vi "test Switch Modules To Scan Mode.vi"(8 "error in (no error)":errorcluster, 11 "TestCase in":refnum<class "Scan Engine cRIO 904x-905x System Tests.lvclass">) -> (0 "error out":errorcluster, 3 "TestCase out":refnum<class "Scan Engine cRIO 904x-905x System Tests.lvclass">)   [LabVIEW 2016, in "Scan Engine cRIO 904x-905x System Tests.lvclass"]
uses:
  Scan Engine cRIO 904x-905x System Tests.lvclass
  <vilib>/nisyscfg/Filter Mode.ctl
  <vilib>/nisyscfg/Save Changes (Hardware).vi
  <vilib>/nisyscfg/Close (Filter).vi
  <vilib>/nisyscfg/Close (System).vi
  <vilib>/nisyscfg/Close (Resources).vi
  <vilib>/addons/_JKI Toolkits/VI Tester/TestCase.llb/TestCase.lvclass
  <vilib>/nisyscfg/nisyscfg.lvlib
  <resource>/objmgr/nisysapi.rc
  <resource>/objmgr/nicriosae.rc
  C:/Program Files (x86)/National Instruments/LabVIEW 2016/vi.lib/addons/_JKI Toolkits/VI Tester/TestCase.llb/TestCase.lvclass
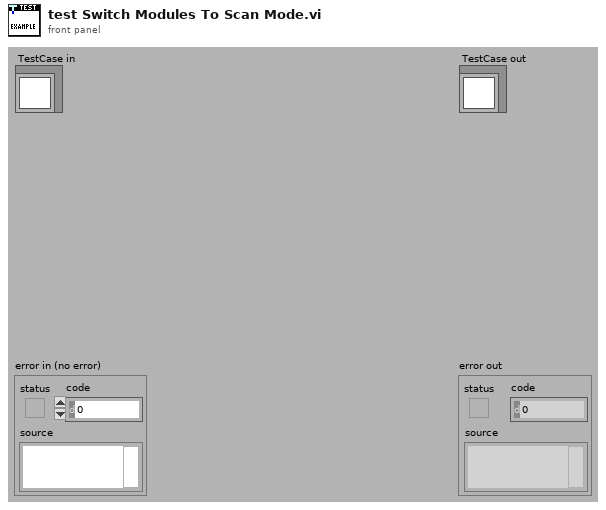
[diagram p1: front panel]
types:
  T1 = cluster{"y":i32, "Devices & Chassis:Bus Specific:cRIO Module Programming Mode":u32}[]
  T2 = typedef "nisyscfg.lvlib/Filter Mode.ctl" = i32
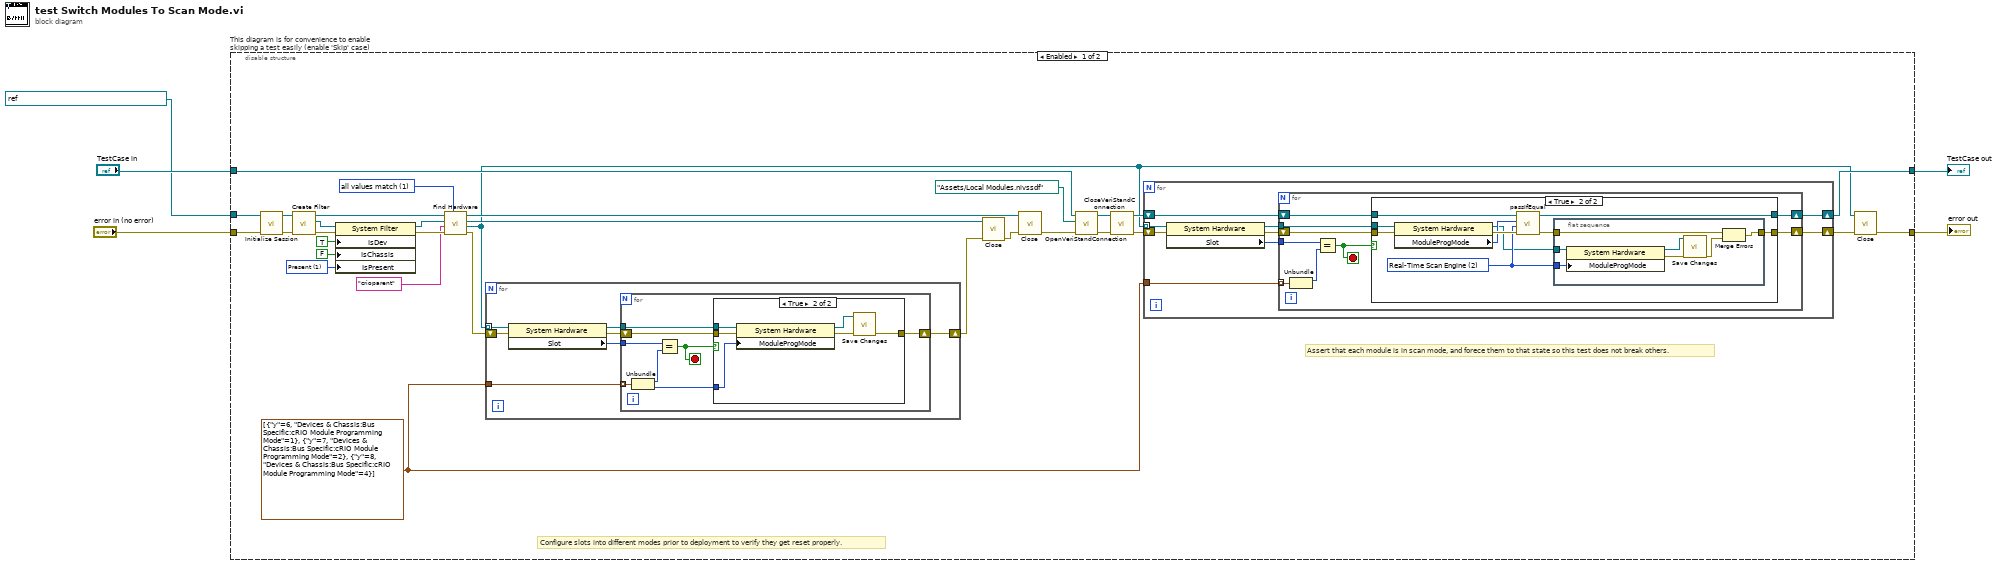
[diagram p0: block diagram]
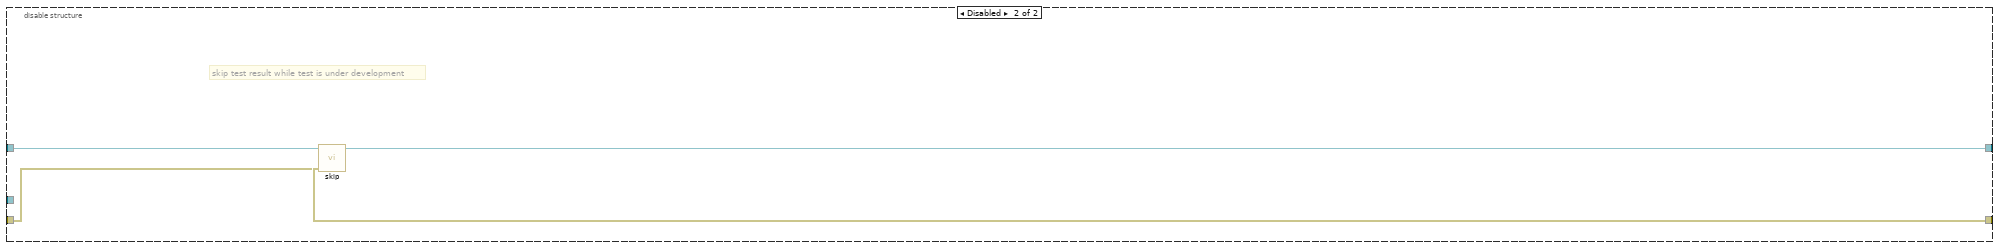
[diagram p4: hidden frame]
diagram:
  n1 = disable-structure "This diagram is for convenience to enable skipping a test easily (enable 'Skip' case)" shown="Enabled" {
    disable-tunnel: "TestCase in" -> [w17 w99]
    disable-tunnel: [w9 w97] -> w2
    disable-tunnel: [w7 w98] -> w4
    disable-tunnel: "error in (no error)" -> [w36 w96]
    disable-tunnel: refnum<k21> "NI-cRIO-9045-01CEEDFB (10.2.64.28)" ("Target (localhost)") -> [w26 _]
    frame Enabled {
      w12 = T1 [{"y"=6, "Devices & Chassis:Bus Specific:cRIO Module Programming Mode"=1}, {"y"=7, "Devices & Chassis:Bus Specific:cRIO Module Programming Mode"=2}, {"y"=8, "Devices & Chassis:Bus Specific:cRIO Module Programming Mode"=4}] ("output cluster")
      w22 = 1 items=["Initializing"=-2, "Unknown"=-1, "Not Present"=0, "Present"=1] ("Devices & Chassis:Is Present")
      w27 = T2 1 items=["all values match"=1, "any value matches"=2, "values do not match"=3, "all properties exist"=4] ("filter mode (all values match)")
      # "Configure slots into different modes prior to deployment to verify they get reset properly."
      # "Assert that each module is in scan mode, and forece them to that state so this test does not break others."
      n2 = call <vilib>:"Initialize Session.vi"("error in (no error)"=w36, "Target (localhost)"=w26) -> ("error out"=w28:errorcluster, "Session out"=w29:refnum<k21>)  [unwired: 8 in]
      n3 = call <vilib>:"Create Filter.vi"("error in (no error)"=w28, "Session in"=w29) -> ("error out"=w35:errorcluster, "Filter out"=w34:refnum<k20>, "Session out"=w33:refnum<k21>)  [unwired: 7 in]
      n4 = property class="System Filter"(reference=w34, error in=w35, "IsDev"=TRUE ("Is Chassis"), "IsChassis"=FALSE ("Is Chassis"), "IsPresent"=w22) -> (reference out=w31:refnum<k20>, error out=w32:errorcluster)
      n5 = call <vilib>:"Find Hardware.vi"("Filter Mode (all values match)"=w27, "error in (no error)"=w32, "Experts"="crioparent", "Filter in"=w31, "Session in"=w33) -> ("error out"=w21:errorcluster, "Resources out"=w6:refnum<k20>[], "Filter out"=w25:refnum<k20>, "Session out"=w19:refnum<k21>)  [unwired: 3 out]
      n6 = for {
        tunnel: w6 -> [w42] mode=indexing
        shift-right: [w37] -> w20
        shift-left: w21 -> [w43]
        tunnel: w12 -> [w40]
        n7 = property class="System Hardware"(reference=w42, error in=w43) -> (reference out=w39:refnum<k20>, error out=w38:errorcluster, "Slot"=w41:i32)
        n8 = for {
          tunnel: w41 -> [w51]
          tunnel: w40 -> [w50] mode=indexing
          tunnel: w39 -> [w47]
          shift-right: [w45] -> w37
          shift-left: w38 -> [w46]
          stop <- w44 stop-if-true
          n9 = Unbundle(w50) -> ("y"=w49:i32, "Devices & Chassis:Bus Specific:cRIO Module Programming Mode"=w48:u32)
          n10 = Equal?(x=w51, y=w49) -> (x = y?=w44:bool)
          n11 = case shown="True" w44 {
            tunnel: w48 -> [_ w58]
            tunnel: w47 -> [_ w57]
            tunnel: w46 -> [w52 w56]
            tunnel: [w52 w53] -> w45
            frame False {
            }
            frame True {
              n12 = property class="System Hardware"(reference=w57, error in=w56, "ModuleProgMode"=w58) -> (reference out=w55:refnum<k20>, error out=w54:errorcluster)
              n13 = call-poly <vilib>:"Save Changes.vi"("error in (no error)"=w54, "Resource in"=w55) -> ("error out"=w53:errorcluster)  [unwired: 6 in, 3 out]
            }
          }
        }
      }
      n14 = call-poly <vilib>:"Close.vi"("error in (no error)"=w20, "Filter in"=w25) -> ("error out"=w18:errorcluster)  [unwired: 9 in]
      n15 = call-poly <vilib>:"Close.vi"("error in (no error)"=w18, "Session in"=w19) -> ("error out"=w16:errorcluster)  [unwired: 9 in]
      n16 = call-dynamic "OpenVeriStandConnection.vi"("error in (no error)"=w16, "System Definition File"=path "Assets/Local Modules.nivssdf", "VeriStand Test Case in"=w17) -> ("error out"=w14:errorcluster, "VeriStand Test Case out"=w15:refnum<class "Scan Engine cRIO 904x-905x System Tests.lvclass">)  [unwired: 7 in]
      n17 = call-dynamic "CloseVeriStandConnection.vi"("error in (no error)"=w14, "VeriStand Test Case in"=w15) -> ("error out"=w11:errorcluster, "VeriStand Test Case out"=w10:refnum<class "Scan Engine cRIO 904x-905x System Tests.lvclass">)  [unwired: 8 in]
      n18 = for {
        tunnel: w6 -> [w66] mode=indexing
        shift-right: [w61] -> w8
        shift-left: w11 -> [w67]
        tunnel: w12 -> [w64]
        shift-right: [w59] -> w9
        shift-left: w10 -> [w60]
        n19 = property class="System Hardware"(reference=w66, error in=w67) -> (reference out=w63:refnum<k20>, error out=w62:errorcluster, "Slot"=w65:i32)
        n20 = for {
          tunnel: w65 -> [w76]
          tunnel: w64 -> [w75] mode=indexing
          tunnel: w63 -> [w73]
          shift-right: [w71] -> w61
          shift-left: w62 -> [w72]
          shift-right: [w68] -> w59
          shift-left: w60 -> [w69]
          stop <- w70 stop-if-true
          n21 = Unbundle(w75) -> ("y"=w74:i32)  [unwired: 1 out]
          n22 = Equal?(x=w76, y=w74) -> (x = y?=w70:bool)
          n23 = case shown="True" w70 {
            tunnel: w73 -> [_ w88]
            tunnel: w72 -> [w78 w87]
            tunnel: [w78 w80] -> w71
            tunnel: w69 -> [w77 w85]
            tunnel: [w77 w84] -> w68
            frame False {
            }
            frame True {
              w82 = u32 2 items=["None"=0, "Real-Time CPU"=1, "Real-Time Scan Engine"=2, "LabVIEW FPGA"=4] ("Devices & Chassis:Bus Specific:cRIO Module Programming Mode")
              n24 = property class="System Hardware"(reference=w88, error in=w87) -> (reference out=w79:refnum<k20>, error out=w86:errorcluster, "ModuleProgMode"=w83:u32)
              n25 = call-dynamic "passIfEqual.vi"("error in (no error)"=w86, "y"=w82, "x"=w83, "TestCase in"=w85) -> ("error out"=w81:errorcluster, "TestCase out"=w84:refnum<class "Scan Engine cRIO 904x-905x System Tests.lvclass">)  [unwired: 6 in]
              n26 = flat-sequence {
                tunnel: w82 -> [w95]
                tunnel: w81 -> [w94]
                tunnel: [w93] -> w80
                tunnel: w79 -> [w92]
                frame #0 {
                  n27 = property class="System Hardware"(reference=w92, "ModuleProgMode"=w95) -> (reference out=w90:refnum<k20>, error out=w91:errorcluster)  [unwired: 1 in]
                  n28 = call-poly <vilib>:"Save Changes.vi"("error in (no error)"=w91, "Resource in"=w90) -> ("error out"=w89:errorcluster)  [unwired: 6 in, 3 out]
                  n29 = Merge Errors(w94, w89) -> (w93:errorcluster)
                }
              }
            }
          }
        }
      }
      n30 = call-poly <vilib>:"Close.vi"("error in (no error)"=w8, "Resources in"=w6) -> ("error out"=w7:errorcluster)  [unwired: 9 in]
    }
    frame Disabled {
      # "skip test result while test is under development"
      n31 = call <vilib>:"skip.vi"("error in (no error)"=w96, "TestCase in"=w99) -> ("error out"=w98:errorcluster, "TestCase out"=w97:refnum<class "Scan Engine cRIO 904x-905x System Tests.lvclass">)  [unwired: 8 in]
    }
  }
  "error out" <- w4
  "TestCase out" <- w2
